vi "Launch Nested.vi"(8 "error in (no error)":errorcluster, 9 "Config Element":refnum<class "VolatusConfigElement.lvclass">, 10 "Nested Module":refnum<class "Module.lvclass">, 11 "Parent in":refnum<class "Module.lvclass">) -> (0 "error out":errorcluster, 2 "MessageQ":refnum<class "MessageQ.lvclass">, 3 "Parent out":refnum<class "Module.lvclass">)   [LabVIEW 2020, in "Volatus.lvlib" / "Module.lvclass"]
uses:
  Module.lvclass
  MessageQ/MessageQ.lvclass
  VolatusConfig/VolatusConfigElement/VolatusConfigElement.lvclass
  Module.lvclass/Module.ctl
  State.ctl
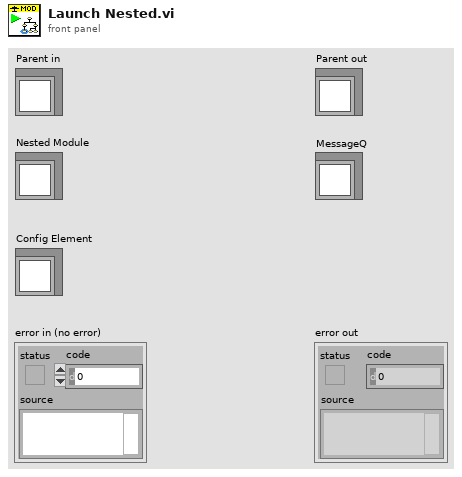
[diagram p1: front panel]
types:
  T1 = typedef "Volatus.lvlib/Module.lvclass/State.ctl" = enum16{"Unknown", "Launched", "Starting", "Running", "Stopping", "Stopped", "Error - Starting", "Error - Run", "Error - Stopping"}
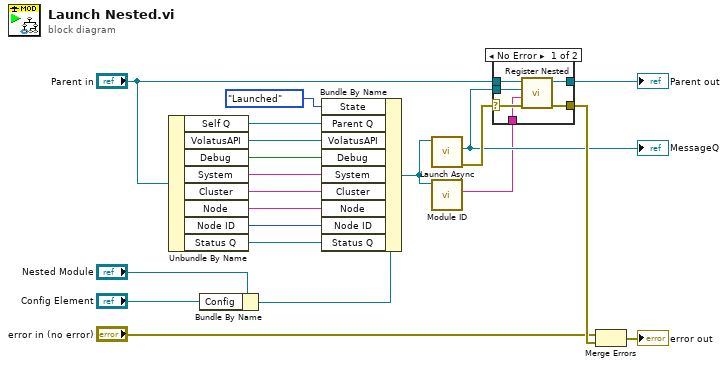
[diagram p0: block diagram]
diagram:
  n1 = Unbundle By Name("Parent in") -> ("Self Q"=w14:refnum<class "MessageQ.lvclass">, "VolatusAPI"=w13:refnum<class "VolatusAPI.lvclass">, "Debug"=w9:bool, "System"=w8:string, "Cluster"=w7:string, "Node"=w6:string, "Node ID"=w5:u32, "Status Q"=w2:refnum<class "MessageQ.lvclass">)
  n2 = Bundle By Name(cluster="Nested Module", "Config"="Config Element") -> (w11:refnum<class "Module.lvclass">)
  n3 = Bundle By Name(cluster=w11, "State"=State."Launched", "Parent Q"=w14, "VolatusAPI"=w13, "Debug"=w9, "System"=w8, "Cluster"=w7, "Node"=w6, "Node ID"=w5, "Status Q"=w2) -> (w4:refnum<class "Module.lvclass">)
  n4 = call "Launch Async.vi"("Module in"=w4) -> ("error out"=w20:errorcluster, "MessageQ"=w12:refnum<class "MessageQ.lvclass">)  [unwired: 9 in]
  "MessageQ" <- w12
  n5 = call-dynamic "Module ID.vi"("Module in"=w4) -> ("Module ID"=w3:string)  [unwired: 10 in]
  n6 = case shown="No Error" w20 {
    selector: w20 -> [w25 w28]
    tunnel: w12 -> [w26 _]
    tunnel: "Parent in" -> [w27 w29]
    tunnel: [w23 w29] -> w16
    tunnel: [w24 w28] -> w21
    tunnel: w3 -> [w22 _]
    frame No Error {
      n7 = call "Register Nested.vi"("error in (no error)"=w25, "Module ID"=w22, "MessageQ"=w26, "Module in"=w27) -> ("error out"=w24:errorcluster, "Module out"=w23:refnum<class "Module.lvclass">)  [unwired: 6 in]
    }
    frame Error {
    }
  }
  "Parent out" <- w16
  n8 = Merge Errors("error in (no error)", w21) -> (→"error out":errorcluster)
